vi "Read Topic Descriptor.vi"(8 "error in (no error)":errorcluster, 9 "timeout_ms":u32=5000, 11 "Topic Full Names":T1) -> (0 "error out":errorcluster, 2 "type_name":string, 3 "descriptor":string)   [LabVIEW 2021, in "Iceoryx.lvlib"]
uses:
  Iceoryx.lvlib
  typedef/Topic Full Names.ctl
  SubVIs/Convert Error Core.vi
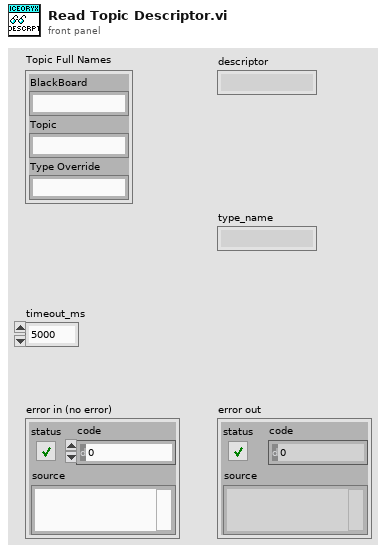
[diagram p1: front panel]
types:
  T1 = typedef "Iceoryx.lvlib/Topic Full Names.ctl" = cluster{"BlackBoard":string, "Topic":string, "Type Override":string}
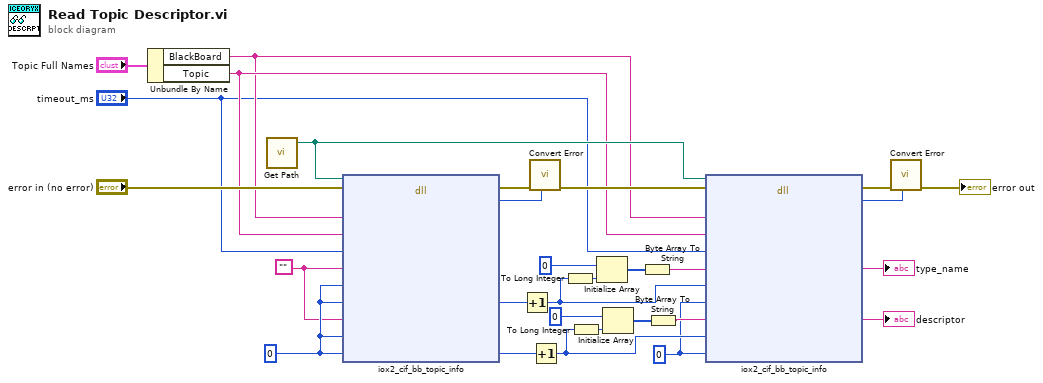
[diagram p0: block diagram]
diagram:
  w6 = u32 0 ("actual")
  w24 = ""
  w25 = u32 0 ("actual")
  n1 = Unbundle By Name("Topic Full Names") -> ("BlackBoard"=w2:string, "Topic"=w3:string)
  n2 = call "Get Path.vi"() -> ("libiox2_cif path"=w19:path)  [unwired: 4 in]
  n3 = dll-call lib="D:/dev/iceoryx2_lvwrapper/dist/iox2_cif.dll" fn="iox2_cif_bb_topic_info"(path in=w19, error in="error in (no error)", "bb_name"=w2, "topic"=w3, "timeout_ms"="timeout_ms", "type_name"=w24, "type_cap"=w25, "type_len"=w25, "descriptor"=w24, "desc_cap"=w25, "desc_len"=w25) -> (error out=w27:errorcluster, "return type"=w26:i32, "type_len"=w18:u32, "desc_len"=w9:u32)  [unwired: 8 in, 1 out]
  n4 = Increment(x=w18) -> (x+1=w16:u32)
  n5 = call "Convert Error.vi"("return type"=w26, "error in (no error)"=w27) -> ("error out"=w21:errorcluster)  [unwired: 9 in]
  n6 = Increment(x=w9) -> (x+1=w7:u32)
  n7 = To Long Integer(number=w16) -> (32bit integer=w15:i32)
  n8 = To Long Integer(number=w7) -> (32bit integer=w11:i32)
  n9 = Initialize Array(u8 0 ("actual"), w15) -> (w14:u8[])
  n10 = Initialize Array(u8 0 ("actual"), w11) -> (w12:u8[])
  n11 = Byte Array To String(unsigned byte array=w14) -> (string=w13:string)
  n12 = Byte Array To String(unsigned byte array=w12) -> (string=w8:string)
  n13 = dll-call lib="D:/dev/iceoryx2_lvwrapper/dist/iox2_cif.dll" fn="iox2_cif_bb_topic_info"(path in=w19, error in=w21, "bb_name"=w2, "topic"=w3, "timeout_ms"="timeout_ms", "type_name"=w13, "type_cap"=w16, "type_len"=w6, "descriptor"=w8, "desc_cap"=w7, "desc_len"=w6) -> (error out=w22:errorcluster, "return type"=w23:i32, "type_name"=→"type_name":string, "descriptor"=→"descriptor":string)  [unwired: 8 in, 1 out]
  n14 = call "Convert Error.vi"("return type"=w23, "error in (no error)"=w22) -> ("error out"=→"error out":errorcluster)  [unwired: 9 in]
